vi "Runtime test.vi"() -> (1 "init error":errorcluster, 2 "correct execution settings":bool, 3 "output lookup error":errorcluster, 4 "input error":errorcluster, 5 "serialization problem":errorcluster, 8 "final error":errorcluster, 9 "output error":errorcluster)   [LabVIEW 2014, in "Daqmx Module tests.lvlib"]
doc: "This VI shows an example for how to test the Runtime functionality of the module. This will need to be modified according to module functionality."
uses:
  Daqmx Module tests.lvlib
  module/execution/Daqmx Module runtime.lvclass
  <vilib>/NI/Tag Bus/dictionary/data dictionary.lvclass/data dictionary.ctl
  <vilib>/NI/Tag Bus/dictionary/lookup polymorphs/locate Boolean.vi
  <vilib>/NI/Tag Bus/dictionary/lookup polymorphs/locate double.vi
  <vilib>/NI/Tag Bus/table/data polymorphs/read many/read Doubles.vi
  <vilib>/NI/Tag Bus/table/data polymorphs/read many/read Booleans.vi
  <vilib>/NI/Tag Bus/dictionary/search/find data index.vi
  <vilib>/NI/Tag Bus/dictionary/search/search string list.vi
  <vilib>/NI/Tag Bus/dictionary/tag not found.vi
  module/configuration/Daqmx Module configuration.lvclass
  <vilib>/NI/Tag Bus/dictionary/data dictionary.lvclass
  <vilib>/NI/Tag Bus/table/data table.lvlib
  <vilib>/NI/Tag Bus/table/data polymorphs/write one/write Double.vi
panel:
  out "Waveform Chart 2":cluster{"[0]":i16, "[1]":i16}(graph)
  in  "stop":bool
  out "Waveform Chart":cluster{"values[0]":dbl, "values[1]":dbl}(graph)
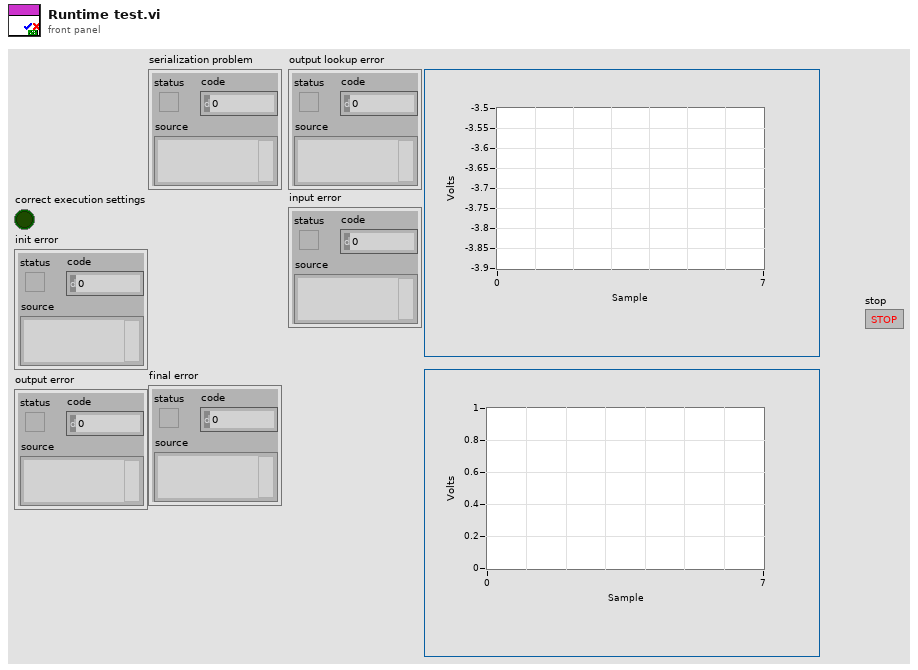
[diagram p1: front panel]
types:
  T1 = typedef "TBM channel.lvclass/data tables.ctl" = cluster{"input data":T2, "processing parameter":T2, "processing result":T2, "output data":T2}
  T2 = typedef "tag bus.lvlib/dictionary table pair.ctl" = cluster{"data dictionary":refnum<class "data dictionary.lvclass">, "data table":T3}
  T3 = typedef "tag bus.lvlib/data table.lvlib/data table.ctl" = cluster{"Double":dbl[], "Single":sgl[], "I64":i64[], "I32":i32[], "I16":i16[], "I8":i8[], "U64":u64[], "U32":u32[], "U16":u16[], "U8":u8[], "Boolean":bool[], "String":string[], "Array of Double":cluster{"DBL Array":dbl[]}[], "Array of Single":cluster{"SGL Array":sgl[]}[], "Array of I64":cluster{"I64 Array":i64[]}[], "Array of I32":cluster{"I32 Array":i32[]}[], "Array of I16":cluster{"I16 Array":i16[]}[], "Array of I8":cluster{"I8 Array":i8[]}[], "Array of U64":cluster{"U64 Array":u64[]}[], "Array of U32":cluster{"U32 Array":u32[]}[], "Array of U16":cluster{"U16 Array":u16[]}[], "Array of U8":cluster{"U8 Array":u8[]}[], "Array of Boolean":cluster{"Boolean Array":bool[]}[], "Array of String":cluster{"String Array":string[]}[]}
  T4 = typedef "TBM module execution interface.lvclass/execution settings.ctl" = cluster{"reads inputs":bool, "processes data":bool, "writes outputs":bool}
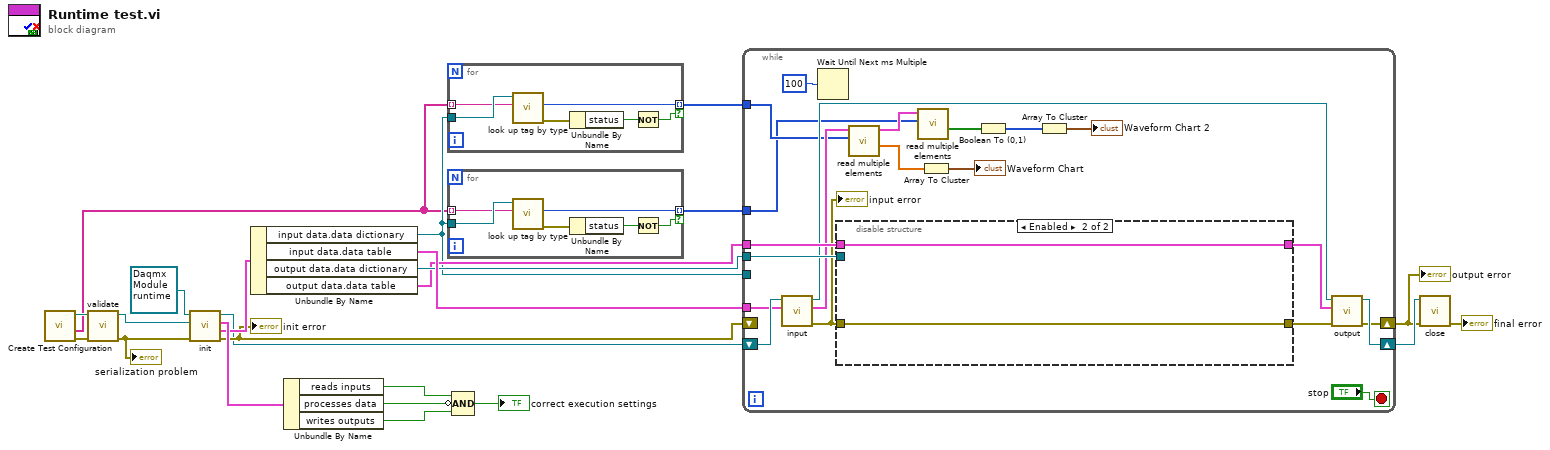
[diagram p0: block diagram]
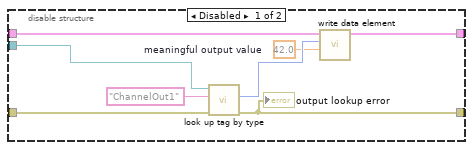
[diagram p2: hidden frame]
diagram:
  n1 = call "Create Test Configuration.vi"() -> ("error out"=w5:errorcluster, "Names"=w2:string[], "Module Configuration"=w6:refnum<class "Daqmx Module configuration.lvclass">)  [unwired: 6 in, 3 out]
  n2 = call-dynamic "validate.vi"("error in"=w5, "Daqmx Module configuration in"=w6) -> ("error out"=w22:errorcluster, "Daqmx Module configuration out"=w21:refnum<class "Daqmx Module configuration.lvclass">)  [unwired: 8 in]
  "serialization problem" <- w22
  n3 = call-dynamic "init.vi"("error in"=w22, "TBM module configuration in"=w21, "Daqmx Module runtime in"=refnum<class "Daqmx Module runtime.lvclass"> refnum ("tag bus configurable plugin module")) -> ("error out"=w14:errorcluster, "data allocations"=w15:T1, "execution settings"=w20:T4, "Daqmx Module runtime out"=w12:refnum<class "Daqmx Module runtime.lvclass">)  [unwired: 5 in]
  "init error" <- w14
  n4 = Unbundle By Name(w15) -> ("input data.data dictionary"=w3:refnum<class "data dictionary.lvclass">, "input data.data table"=w13:T3, "output data.data dictionary"=w11:refnum<class "data dictionary.lvclass">, "output data.data table"=w10:T3)
  n5 = Unbundle By Name(w20) -> ("reads inputs"=w17:bool, "processes data"=w19:bool, "writes outputs"=w18:bool)
  n6 = for {
    tunnel: w3 -> [w29]
    tunnel: w2 -> [w28] mode=indexing
    tunnel: [w27] -> w4 mode=indexing if=w24
    n7 = call-poly <vilib>:"look up tag by type.vi"("name"=w28, "data dictionary in"=w29) -> ("error out"=w26:errorcluster, "index"=w27:i32)  [unwired: 7 in, 1 out]
    n8 = Unbundle By Name(w26) -> ("status"=w25:bool)
    n9 = Not(x=w25) -> (.not. x?=w24:bool)
  }
  n10 = for {
    tunnel: w3 -> [w35]
    tunnel: w2 -> [w34] mode=indexing
    tunnel: [w33] -> w1 mode=indexing if=w30
    n11 = call-poly <vilib>:"look up tag by type.vi"("name"=w34, "data dictionary in"=w35) -> ("error out"=w32:errorcluster, "index"=w33:i32)  [unwired: 7 in, 1 out]
    n12 = Unbundle By Name(w32) -> ("status"=w31:bool)
    n13 = Not(x=w31) -> (.not. x?=w30:bool)
  }
  n14 = Compound Arithmetic op=AND(w17, invert w19, w18) -> (→"correct execution settings":bool)
  n15 = while {
    tunnel: w3 -> [_]
    tunnel: w13 -> [w45]
    tunnel: w11 -> [w55]
    tunnel: w10 -> [w54]
    shift-right: [w48] -> w8
    shift-left: w14 -> [_]
    shift-right: [w49] -> w9
    shift-left: w12 -> [w56]
    tunnel: w4 -> [w43]
    tunnel: w1 -> [w36]
    stop <- "stop" stop-if-true
    n16 = call-dynamic "input.vi"("data table in"=w45, "Daqmx Module runtime in"=w56) -> ("error out"=w53:errorcluster, "data table out"=w44:T3, "Daqmx Module runtime out"=w51:refnum<class "Daqmx Module runtime.lvclass">)  [unwired: 7 in]
    "input error" <- w53
    n17 = Wait Until Next ms Multiple(millisecond multiple=u32 100) -> ()  [unwired: 1 out]
    n18 = disable-structure shown="Enabled" {
      disable-tunnel: w55 -> [w64 _]
      disable-tunnel: w54 -> [w61 w65]
      disable-tunnel: w53 -> [w60 w66]
      disable-tunnel: [w58 w66] -> w52
      disable-tunnel: [w57 w65] -> w50
      frame Disabled {
        w59 = 42.0  # meaningful output value
        n19 = call-poly <vilib>:"look up tag by type.vi"("error in"=w60, "name"="ChannelOut1" ("channel name"), "data dictionary in"=w64) -> ("error out"=w58:errorcluster, "index"=w62:i32)  [unwired: 6 in, 1 out]
        "output lookup error" <- w58
        n20 = call-poly <vilib>:"write data element.vi"("value"=w59, "index"=w62, "data table in"=w61) -> ("data table out"=w57:T3)  [unwired: 8 in]
      }
      frame Enabled {
      }
    }
    n21 = call-poly <vilib>:"read multiple elements.vi"("indices"=w43, "data table in"=w44) -> ("values"=w42:dbl[], "data table out"=w40:T3)  [unwired: 8 in]
    n22 = call-poly <vilib>:"read multiple elements.vi"("indices"=w36, "data table in"=w40) -> ("values"=w39:bool[])  [unwired: 8 in, 1 out]
    n23 = Array To Cluster(array=w42) -> (cluster=→"Waveform Chart":cluster{"values[0]":dbl, "values[1]":dbl})
    n24 = Boolean To (0,1)(Boolean=w39) -> (0, 1=w38:i16[])
    n25 = Array To Cluster(array=w38) -> (cluster=→"Waveform Chart 2":cluster{"[0]":i16, "[1]":i16})
    n26 = call-dynamic "output.vi"("error in"=w52, "data table in"=w50, "Daqmx Module runtime in"=w51) -> ("error out"=w48:errorcluster, "Daqmx Module runtime out"=w49:refnum<class "Daqmx Module runtime.lvclass">)  [unwired: 6 in, 1 out]
  }
  "output error" <- w8
  n27 = call-dynamic "close.vi"("error in"=w8, "Daqmx Module runtime in"=w9) -> ("error out"=→"final error":errorcluster)  [unwired: 9 in]
